vi "LV Type To JSON Schema.vi"(8 "error in":errorcluster, 11 "type":variant) -> (0 "error out":errorcluster, 3 "JSON Schema":string)   [LabVIEW 2020, in "MCP Server.lvlib"]
doc: "Builds the JSON Schema of a LabVIEW type, for tools/list. Wire any value of the type into type. Numbers are integer or number, Booleans boolean, strings and paths string, timestamps string with format date-time (ISO 8601, which is what tools/call accepts for them), enums string with their item names as enum. An array of N dimensions is N nested levels of {\"type\":\"array\",\"items\":...} around the schema of its element. A cluster is an object whose properties are its elements, named by their labels exactly as tools/call matches them. A type with no JSON equivalent (variant, waveform, refnum, complex number and so on) is {}, which allows any value, so an array of it still says what its items are. Nested arrays and clusters are described to any depth."
uses:
  MCP Server.lvlib
  da39a3ec-8b23-4645-ae79-018f8cedae49.vi
  <vilib>/JDP Science/JSONtext/support/Format JSON Object.vi
  <vilib>/JDP Science/JSONtext/Variant to JSON Text.vi
  <vilib>/JDP Science/JSONtext/LVClass Serializer/JSONtext LVClass Serializer.lvclass
  <vilib>/Utility/Data Type/NI_Data Type.lvlib
  <vilib>/JDP Science/JSONtext/JSONtext.lvlib
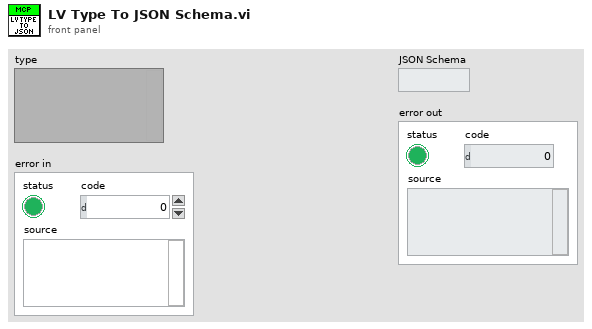
[diagram p1: front panel]
types:
  T1 = typedef "NI_Data Type.lvlib/Data Type.ctl" = enum8{"Invalid Type", "Void", "I8", "I16", "I32", "I64", "U8", "U16", "U32", "U64", "Single Float", "Double Float", "Extended Float", "Single Complex", "Double Complex", "Extended Complex", "Enum U8", "Enum U16", "Enum U32", "Enum U64", "Single Float With Unit", "Double Float With Unit", "Extended Float With Unit", "Single Complex with Unit", "Double Complex with Unit", "Extended Complex with Unit", "Boolean", "String", "Path", "Picture", "Tag", "Array", "Cluster", "Variant", "LV Variant", "Waveform", "Timestamp", "Digital Waveform", "Digital Data", "ExpressData", "Refnum", "External Data", "VI", "Poly VI", "LabVIEW Class Instance", "Fixed Point", "Set Collection", "Map Collection"}
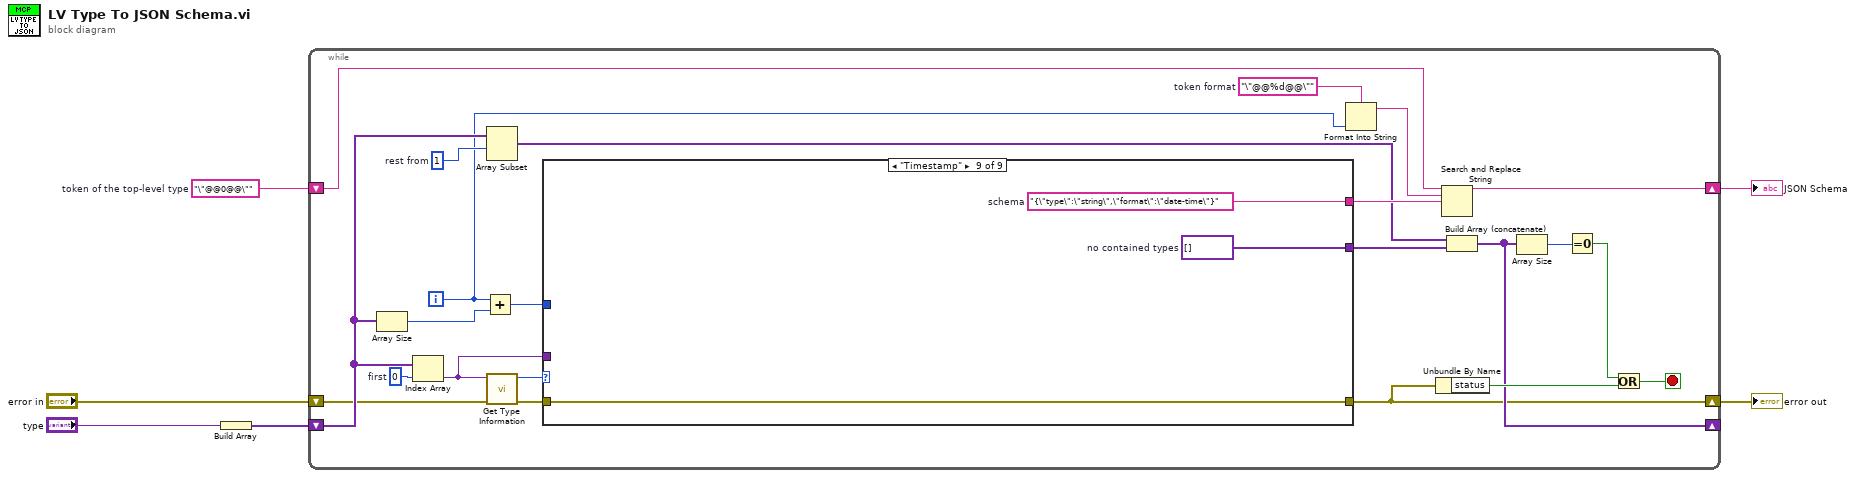
[diagram p0: block diagram]
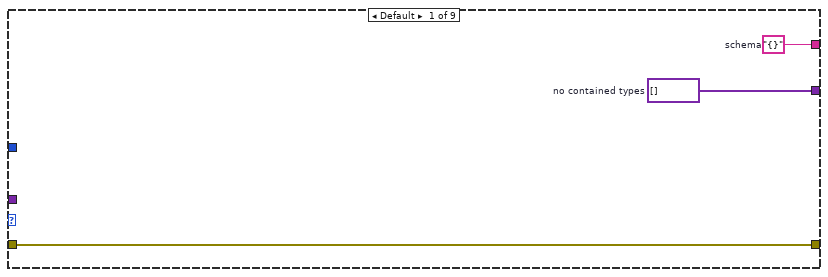
[diagram p2: hidden frame]
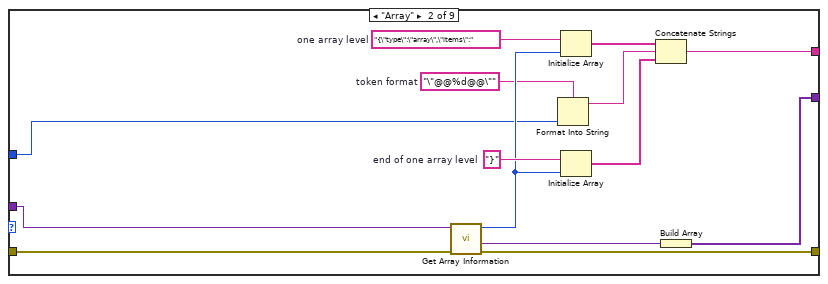
[diagram p3: hidden frame]
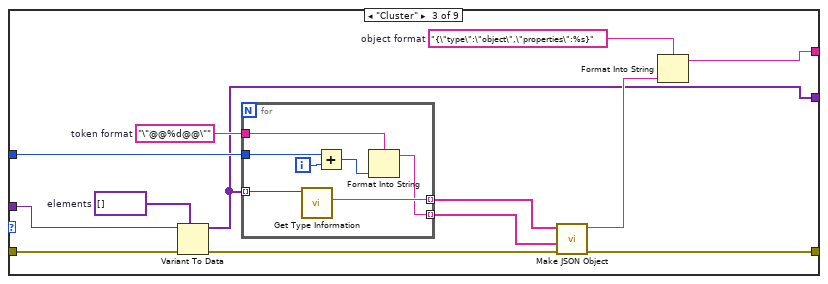
[diagram p4: hidden frame]
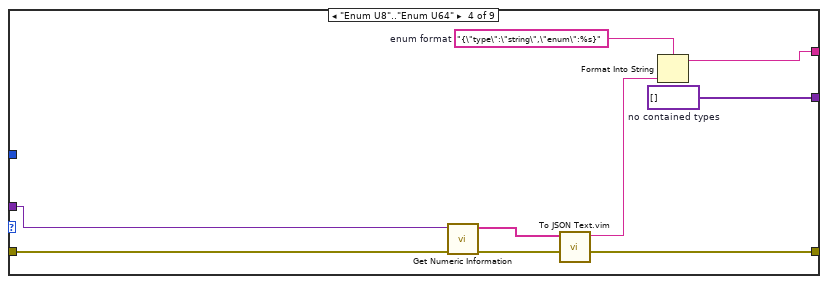
[diagram p5: hidden frame]
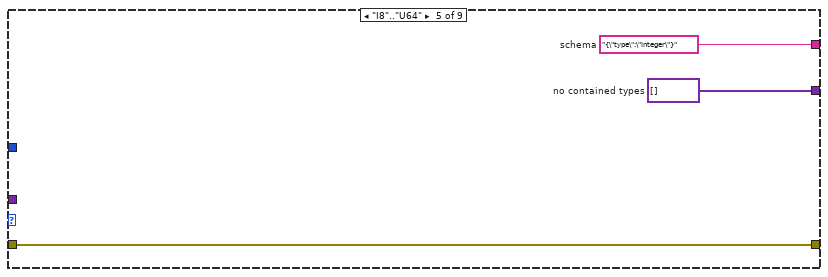
[diagram p6: hidden frame]
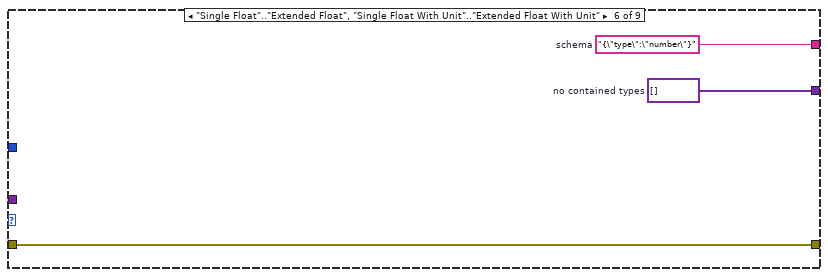
[diagram p7: hidden frame]
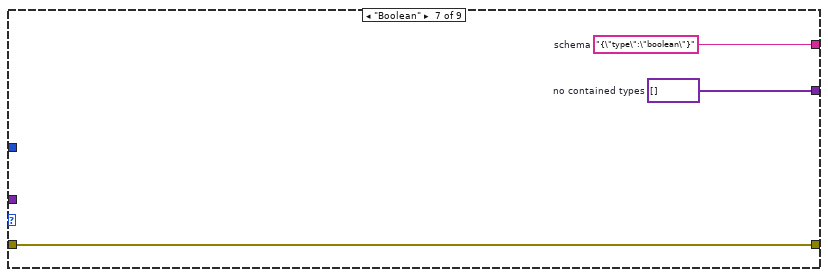
[diagram p8: hidden frame]
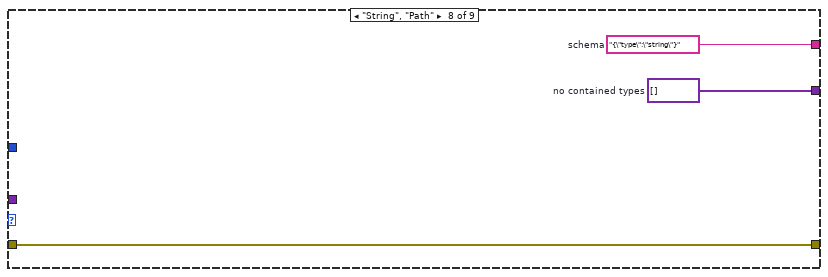
[diagram p9: hidden frame]
diagram:
  w4 = "\"@@0@@\""  # token of the top-level type
  n1 = Build Array("type") -> (w5:variant[])
  n2 = while {
    shift-right: [w13] -> _
    shift-left: w5 -> [w12]
    shift-right: [w11] -> w2
    shift-left: w4 -> [w10]
    shift-right: [w9] -> w1
    shift-left: "error in" -> [w8]
    i -> [w7]
    stop <- w14 stop-if-true
    w26 = "\"@@%d@@\""  # token format
    w28 = 1  # rest from
    w29 = 0  # first
    n3 = Array Size(array=w12) -> (size(s)=w27:i32)
    n4 = Index Array(array=w12, index=w29) -> (element=w25:variant)
    n5 = Add(x=w7, y=w27) -> (x+y=w24:i32)
    n6 = Array Subset(array=w12, index=w28) -> (w19:variant[])  [unwired: 1 in]
    n7 = call <vilib>:"Get Type Information.vi"("error in (no error)"=w8, "variant"=w25) -> ("error out"=w23:errorcluster, "type"=w22:T1)  [unwired: 5 in, 3 out]
    n8 = case shown="\"Timestamp\"" w22 {
      tunnel: w25 -> [_ w46 w59 w75 _ _ _ _ _]
      tunnel: w24 -> [_ w40 w56 _ _ _ _ _ _]
      tunnel: w23 -> [w30 w45 w58 w74 w76 w79 w82 w85 w88]
      tunnel: [w32 w35 w49 w69 w78 w81 w84 w87 w90] -> w20
      tunnel: [w31 w34 w48 w68 w77 w80 w83 w86 w89] -> w18
      tunnel: [w30 w33 w47 w67 w76 w79 w82 w85 w88] -> w9
      frame Default {
        w31 = variant[] []  # no contained types
        w32 = "{}"  # schema
      }
      frame "Array" {
        w41 = "\"@@%d@@\""  # token format
        w43 = "}"  # end of one array level
        w44 = "{\"type\":\"array\",\"items\":"  # one array level
        n9 = call <vilib>:"Get Array Information.vi"("error in (no error)"=w45, "variant"=w46) -> ("error out"=w33:errorcluster, "array element data type"=w36:variant, "number of dimensions"=w42:i32)  [unwired: 6 in, 1 out]
        n10 = Format Into String(format string=w41, w40) -> (resulting string=w38:string)  [unwired: 2 in, 1 out]
        n11 = Initialize Array(w44, w42) -> (w39:string[])
        n12 = Initialize Array(w43, w42) -> (w37:string[])
        n13 = Concatenate Strings(w39, w38, w37) -> (w35:string)
        n14 = Build Array(w36) -> (w34:variant[])
      }
      frame "Cluster" {
        w51 = "{\"type\":\"object\",\"properties\":%s}"  # object format
        w55 = "\"@@%d@@\""  # token format
        w57 = variant[] []  # elements
        n15 = Variant To Data(error in=w58, type=w57, Variant=w59) -> (data=w48:variant[], error out=w52:errorcluster)
        n16 = for {
          tunnel: w48 -> [w66] mode=indexing
          tunnel: w56 -> [w65]
          tunnel: w55 -> [w64]
          tunnel: [w62] -> w54 mode=indexing
          tunnel: [w61] -> w53 mode=indexing
          i -> [w60]
          n17 = call <vilib>:"Get Type Information.vi"("variant"=w66) -> ("name"=w62:string)  [unwired: 6 in, 4 out]
          n18 = Add(x=w65, y=w60) -> (x+y=w63:i32)
          n19 = Format Into String(format string=w64, w63) -> (resulting string=w61:string)  [unwired: 2 in, 1 out]
        }
        n20 = call <vilib>:"Make JSON Object.vi"("error in (no error)"=w52, "JSON Items"=w53, "Item Names"=w54) -> ("error out"=w47:errorcluster, "<JSON>"=w50:string)  [unwired: 7 in]
        n21 = Format Into String(format string=w51, w50) -> (resulting string=w49:string)  [unwired: 2 in, 1 out]
      }
      frame "Enum U8".."Enum U64" {
        w68 = variant[] []  # no contained types
        w71 = "{\"type\":\"string\",\"enum\":%s}"  # enum format
        n22 = call <vilib>:"Get Numeric Information.vi"("error in (no error)"=w74, "variant"=w75) -> ("error out"=w72:errorcluster, "enum names"=w73:string[])  [unwired: 6 in, 2 out]
        n23 = call "To JSON Text.vim"("error in (no error)"=w72, "Anything"=w73) -> ("error out"=w67:errorcluster, "<JSON>"=w70:string)  [unwired: 8 in]
        n24 = Format Into String(format string=w71, w70) -> (resulting string=w69:string)  [unwired: 2 in, 1 out]
      }
      frame "I8".."U64" {
        w77 = variant[] []  # no contained types
        w78 = "{\"type\":\"integer\"}"  # schema
      }
      frame "Single Float".."Extended Float", "Single Float With Unit".."Extended Float With Unit" {
        w80 = variant[] []  # no contained types
        w81 = "{\"type\":\"number\"}"  # schema
      }
      frame "Boolean" {
        w83 = variant[] []  # no contained types
        w84 = "{\"type\":\"boolean\"}"  # schema
      }
      frame "String", "Path" {
        w86 = variant[] []  # no contained types
        w87 = "{\"type\":\"string\"}"  # schema
      }
      frame "Timestamp" {
        w89 = variant[] []  # no contained types
        w90 = "{\"type\":\"string\",\"format\":\"date-time\"}"  # schema
      }
    }
    n25 = Format Into String(format string=w26, w7) -> (resulting string=w21:string)  [unwired: 2 in, 1 out]
    n26 = Unbundle By Name(w9) -> ("status"=w15:bool)
    n27 = Search and Replace String(input string=w10, search string=w21, replace string=w20) -> (result string=w11:string)  [unwired: 5 in, 3 out]
    n28 = Build Array (concatenate)(w19, w18) -> (w13:variant[])
    n29 = Array Size(array=w13) -> (size(s)=w17:i32)
    n30 = Equal To 0?(x=w17) -> (x = 0?=w16:bool)
    n31 = Or(x=w16, y=w15) -> (x .or. y?=w14:bool)
  }
  "JSON Schema" <- w2
  "error out" <- w1
